vi "String Parsing Implementation.vi"(8 "error in (no error)":errorcluster, 11 "class path":path) -> (0 "error out":errorcluster, 3 "Array":path[](array[path]))   [LabVIEW 2020, in "Test Method Finding Test.lvclass"]
uses:
  Test Method Finding Test.lvclass
  Test Method Finding Test.lvclass/Test Method Finding Test.ctl
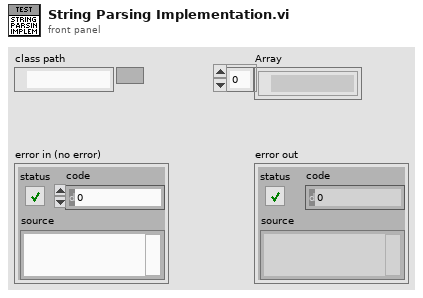
[diagram p1: front panel]
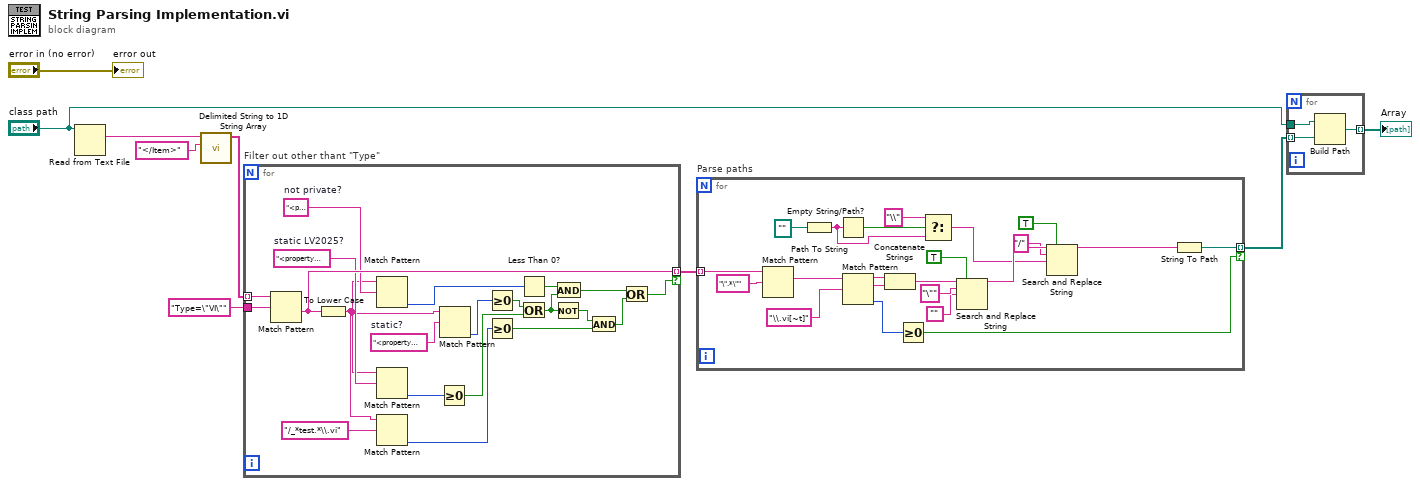
[diagram p0: block diagram]
diagram:
  n1 = Read from Text File(file (use dialog)="class path") -> (text=w8:string)  [unwired: 3 in, 3 out]
  n2 = call <vilib>:"Delimited String to 1D String Array.vi"("delimiter"="</Item>" ("regular expression"), "delimited string"=w8) -> ("string array"=w1:string[])  [unwired: 9 in]
  n3 = for "Filter out other thant \"Type\"" {
    tunnel: w1 -> [w30] mode=indexing
    tunnel: [w25] -> w3 mode=indexing if=w10
    tunnel: "Type=\"VI\"" ("regular expression") -> [w29]
    w14 = "<property name=\"ni.classitem.invokeusage\" type=\"uint\">0"  # static LV2025?
    w24 = "<property name=\"ni.classitem.methodscope\" type=\"uint\">2"  # not private?
    w28 = "<property name=\"ni.classitem.isstaticmethod\" type=\"bool\">true"  # static?
    n4 = Match Pattern(string=w30, regular expression=w29) -> (after substring=w25:string)  [unwired: 1 in, 3 out]
    n5 = To Lower Case(string=w25) -> (all lower case string=w11:string)
    n6 = Match Pattern(string=w11, regular expression=w24) -> (offset past match=w26:i32)  [unwired: 1 in, 3 out]
    n7 = Match Pattern(string=w11, regular expression=w14) -> (offset past match=w15:i32)  [unwired: 1 in, 3 out]
    n8 = Match Pattern(string=w11, regular expression="/_*test.*\\.vi") -> (offset past match=w21:i32)  [unwired: 1 in, 3 out]
    n9 = Greater Or Equal To 0?(x=w15) -> (x >= 0?=w12:bool)
    n10 = Match Pattern(string=w11, regular expression=w28) -> (offset past match=w27:i32)  [unwired: 1 in, 3 out]
    n11 = Greater Or Equal To 0?(x=w27) -> (x >= 0?=w20:bool)
    n12 = Greater Or Equal To 0?(x=w21) -> (x >= 0?=w18:bool)
    n13 = Less Than 0?(x=w26) -> (x < 0?=w23:bool)
    n14 = Or(x=w20, y=w12) -> (x .or. y?=w13:bool)
    n15 = Not(x=w13) -> (.not. x?=w19:bool)
    n16 = And(x=w23, y=w13) -> (x .and. y?=w17:bool)
    n17 = And(x=w19, y=w18) -> (x .and. y?=w16:bool)
    n18 = Or(x=w17, y=w16) -> (x .or. y?=w10:bool)
  }
  n19 = for "Parse paths" {
    tunnel: w3 -> [w52] mode=indexing
    tunnel: [w47] -> w6 mode=indexing if=w38
    n20 = Match Pattern(string=w52, regular expression="\".*\"") -> (match substring=w42:string)  [unwired: 1 in, 3 out]
    n21 = Path To String(path=path "") -> (string=w34:string)
    n22 = Empty String/Path?(string/path=w34) -> (empty?=w36:bool)
    n23 = Match Pattern(string=w42, regular expression="\\.vi[~t]") -> (before substring=w44:string, match substring=w43:string, offset past match=w39:i32)  [unwired: 1 in, 1 out]
    n24 = Concatenate Strings(w44, w43) -> (w41:string)
    n25 = Greater Or Equal To 0?(x=w39) -> (x >= 0?=w38:bool)
    n26 = Select(t="\\" ("search string"), s=w36, f=w34) -> (s? t:f=w33:string)
    n27 = Search and Replace String(replace all?=TRUE ("replace all? (F)"), input string=w41, search string="\"", replace string="") -> (result string=w46:string)  [unwired: 4 in, 3 out]
    n28 = Search and Replace String(replace all?=TRUE ("replace all? (F)"), input string=w46, search string="/", replace string=w33) -> (result string=w40:string)  [unwired: 4 in, 3 out]
    n29 = String To Path(string=w40) -> (path=w47:path)
  }
  n30 = for {
    tunnel: "class path" -> [w55]
    tunnel: w6 -> [w54] mode=indexing
    tunnel: [w53] -> w5 mode=indexing
    n31 = Build Path(base path=w55, name or relative path=w54) -> (appended path=w53:path)
  }
  "Array" <- w5
  "error out" <- "error in (no error)"
